vi "UpdateUserTable.vi"(7 "Login-UI.lvlib:PwdMgr.lvclass":refnum<class "PwdMgr.lvclass">, 8 "Error in":errorcluster caption="Error in (no error)", 11 "User Table":refnum<vi>) -> (0 "error out":errorcluster)   [LabVIEW 2020, in "Login-UI.lvlib"]
uses:
  Login-UI.lvlib
  PwdMgr/PwdMgr.lvclass
  <userlib>/NEVSTOP-Programming-Palette/Configuration/ClusterCfgTable/ClusterCfgTable_nevstop.lvlib
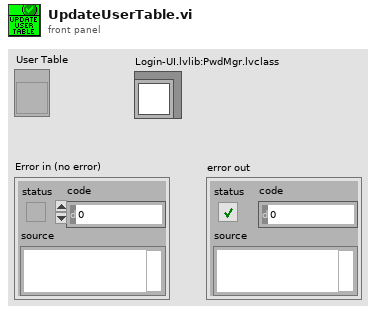
[diagram p1: front panel]
types:
  T1 = typedef "Login-UI.lvlib/User-Info.ctl" = cluster{"UserName":string, "Password":string, "Role":T2}
  T2 = typedef "Login-UI.lvlib/User-Role.ctl" = enum16{"INVALID", "Operator", "Engineer", "Admin", "Anonymous"}
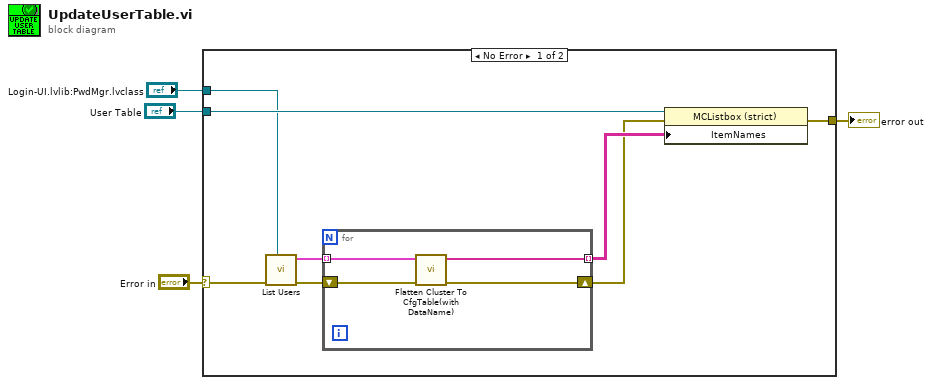
[diagram p0: block diagram]
diagram:
  n1 = case shown="No Error" "Error in" {
    selector: "Error in" -> [w7 w17]
    tunnel: "User Table" -> [w12 _]
    tunnel: [w6 w17] -> w2
    tunnel: "Login-UI.lvlib:PwdMgr.lvclass" -> [w5 _]
    frame No Error {
      n2 = call-dynamic "List Users.vi"("PwdMgr in"=w5, "error in (no error)"=w7) -> ("error out"=w9:errorcluster, "Array"=w11:T1[])  [unwired: 8 in]
      n3 = for {
        tunnel: w11 -> [w16] mode=indexing
        tunnel: [w15] -> w10 mode=indexing
        shift-right: [w13] -> w8
        shift-left: w9 -> [w14]
        n4 = call <userlib>:"Flatten Cluster To CfgTable(with DataName).vi"("error in (no error)"=w14, "Cluster Configuration Typedef"=w16) -> ("error out"=w13:errorcluster, "CfgTable Row"=w15:string[])  [unwired: 7 in, 1 out]
      }
      n5 = property class="MCListbox (strict)"(reference=w12, error in=w8, "ItemNames"=w10) -> (error out=w6:errorcluster)  [unwired: 1 out]
    }
    frame Error {
    }
  }
  "error out" <- w2
